vi "RDB Create Objects.vi"(8 "error in (no error)":errorcluster, 10 "Container ID":string="RDB Reference", 11 "RDB Data Receive":T1) -> (0 "error out":errorcluster, 3 "RDB Reference":refnum<class "DataContainer.lvclass">)   [LabVIEW 2023, in "RDB.lvlib"]
uses:
  RDB.lvlib
  System Explorer/RDB Data.ctl
  RDB Player Object.ctl
  DataContainer/DataContainer.lvclass
  <vilib>/xnet/xnet.llb/XNET Frame FlexRay.ctl
  <vilib>/xnet/xnet.llb/XNET Frame Type FlexRay.ctl
  <vilib>/xnet/xnet.llb/XNET String To IO Name (Signal).vi
  <vilib>/xnet/xnet.llb/XNET Create Session (Conversion).vi
  <resource>/objmgr/xnet.rc
  Shared/Vires VTD Shared.lvlib
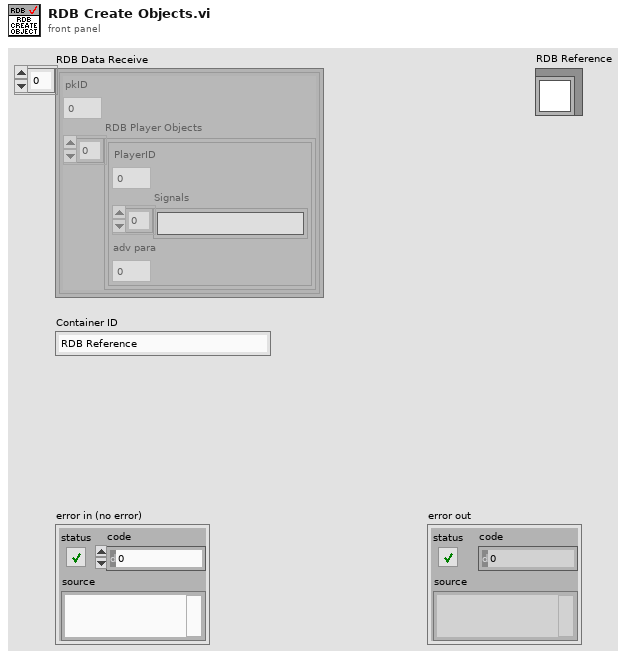
[diagram p1: front panel]
types:
  T1 = typedef "Vires VTD Shared.lvlib/RDB Data.ctl" = cluster{"pkID":i32, "RDB Player Objects":T2[]}[]
  T2 = typedef "RDB.lvlib/RDB Player Object.ctl" = cluster{"PlayerID":i32, "Signals":string[], "adv para":i32}
  T3 = typedef "XNET Frame FlexRay.ctl" = cluster{"timestamp":timestamp, "payload":u8[], "slot":u16, "type":T4, "cycle count":u8, "startup?":bool, "sync?":bool, "preamble?":bool, "ch A":bool, "ch B":bool, "echo?":bool}
  T4 = typedef "XNET Frame Type FlexRay.ctl" = u8
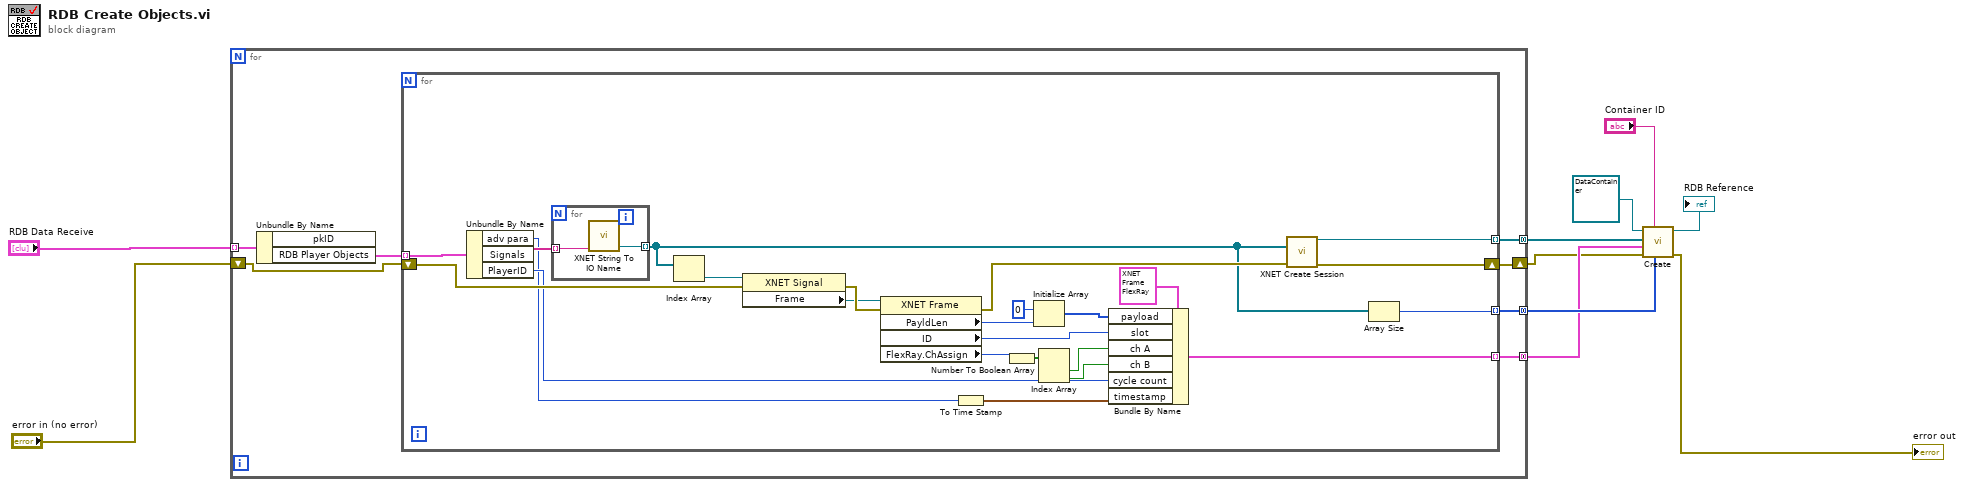
[diagram p0: block diagram]
diagram:
  n1 = for {
    tunnel: "RDB Data Receive" -> [w17] mode=indexing
    shift-right: [w15] -> w3
    shift-left: "error in (no error)" -> [w14]
    tunnel: [w12] -> w6 mode=concatenating
    tunnel: [w13] -> w5 mode=concatenating
    tunnel: [w11] -> w8 mode=concatenating
    n2 = Unbundle By Name(w17) -> ("RDB Player Objects"=w16:T2[])  [unwired: 1 out]
    n3 = for {
      tunnel: w16 -> [w41] mode=indexing
      shift-right: [w40] -> w15
      shift-left: w14 -> [w39]
      tunnel: [w24] -> w13 mode=indexing
      tunnel: [w20] -> w12 mode=indexing
      tunnel: [w18] -> w11 mode=indexing
      n4 = Unbundle By Name(w41) -> ("adv para"=w22:i32, "Signals"=w37:string[], "PlayerID"=w25:i32)
      n5 = for {
        tunnel: w37 -> [w42] mode=indexing
        tunnel: [w43] -> w19 mode=indexing
        n6 = call-poly <vilib>:"XNET String To IO Name.vi"("string"=w42) -> ("XNET Signal"=w43:refnum<k21>)  [unwired: 4 out]
      }
      n7 = Index Array(array=w19) -> (element=w26:refnum<k21>)  [unwired: 1 in]
      n8 = property class="XNET Signal"(reference=w26, error in=w39) -> (error out=w36:errorcluster, "Frame"=w35:refnum<k21>)  [unwired: 1 out]
      n9 = property class="XNET Frame"(reference=w35, error in=w36) -> (error out=w38:errorcluster, "PayldLen"=w28:u32, "ID"=w30:u32, "FlexRay.ChAssign"=w31:u32)  [unwired: 1 out]
      n10 = To Time Stamp(1:w22) -> (0:w21:timestamp)
      n11 = Number To Boolean Array(number=w31) -> (Boolean array=w27:bool[])
      n12 = Initialize Array(0 ("element"), w28) -> (w29:i32[])
      n13 = Index Array(array=w27) -> (element #1=w32:bool, element #2=w33:bool)  [unwired: 2 in]
      n14 = Bundle By Name(cluster=T3 {"timestamp"=timestamp(0 s since 1904-01-01), "payload"=[], "slot"=1, "type"=32, "cycle count"=0, "startup?"=FALSE, "sync?"=FALSE, "preamble?"=FALSE, "ch A"=FALSE, "ch B"=FALSE, "echo?"=FALSE} ("FlexRay frame"), "payload"=w29, "slot"=w30, "ch A"=w32, "ch B"=w33, "cycle count"=w25, "timestamp"=w21) -> (w24:T3)
      n15 = call-poly <vilib>:"XNET Create Session.vi"("signal list"=w19, "error in (no error)"=w38) -> ("session out"=w20:refnum<k21>, "error out"=w40:errorcluster)  [unwired: 12 in]
      n16 = Array Size(array=w19) -> (size(s)=w18:i32)
    }
  }
  n17 = call-dynamic "Create.vi"("noSignals"=w8, "Container ID"="Container ID", "error in (no error)"=w3, "Package Data"=w5, "Conversion References"=w6, "DataContainer in"=refnum<class "DataContainer.lvclass"> refnum) -> ("error out"=→"error out":errorcluster, "DataContainer out"=→"RDB Reference":refnum<class "DataContainer.lvclass">)  [unwired: 4 in]
